vi "GetVarVal.vi"(8 "error in (no error)":errorcluster, 10 "varName":string, 11 "muExpr in":refnum<class "mupExpr.lvclass">) -> (0 "error out":errorcluster, 2 "varValue":dbl, 3 "muExpr out":refnum<class "mupExpr.lvclass">)   [LabVIEW 2018, in "mupExpr.lvclass"]
uses:
  mupExpr.lvclass
  mupExpr.lvclass/mupExpr.ctl
  <vilib>/Utility/error.llb/Error Cluster From Error Code.vi
  <vilib>/ErrorRing/Error Ring.xnode
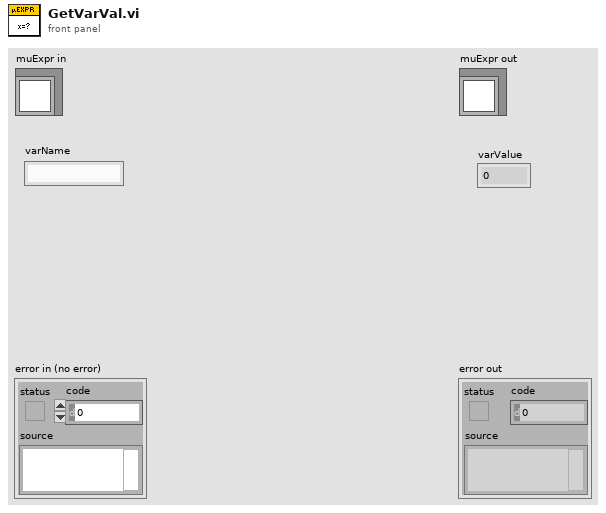
[diagram p1: front panel]
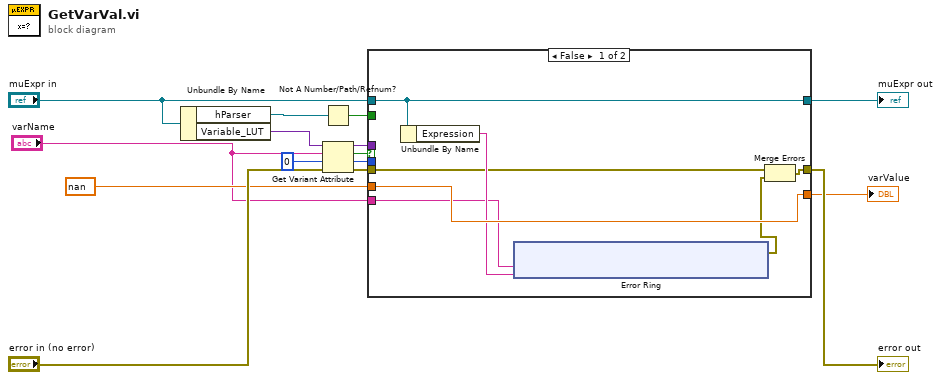
[diagram p0: block diagram]
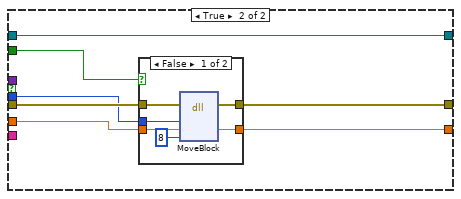
[diagram p2: hidden frame]
diagram:
  n1 = Unbundle By Name("muExpr in") -> ("hParser"=w2:refnum<data-value>, "Variable_LUT"=w8:variant)
  n2 = Not A Number/Path/Refnum?(number/path/refnum=w2) -> (NaN/Path/Refnum?=w1:bool)
  n3 = Get Variant Attribute(Variant=w8, name="varName", default value (empty Variant)=u64 0 ("pd"), error in="error in (no error)") -> (duplicate Variant=w3:variant, found=w4:bool, value=w5:u64, error out=w7:errorcluster)
  n4 = case shown="False" w4 {
    tunnel: w7 -> [w18 w36]
    tunnel: nan ("varValue") -> [w21 w34]
    tunnel: w5 -> [_ w33]
    tunnel: [w17 w35] -> w14
    tunnel: "varName" -> [w19 _]
    tunnel: "muExpr in" -> [w22 w37]
    tunnel: w3 -> [_ _]
    tunnel: [w22 w37] -> w12
    tunnel: [w21 w32] -> w9
    tunnel: w1 -> [_ w31]
    frame False {
      n5 = Unbundle By Name(w22) -> ("Expression"=w20:string)
      n6 = xnode "Error Ring"("parameter 0"=w19, "parameter 1"=w20) -> ("error out"=w16:errorcluster)
      n7 = Merge Errors(w18, w16) -> (w17:errorcluster)
    }
    frame True {
      n8 = case shown="False" w31 {
        tunnel: w36 -> [w42 w45]
        tunnel: [w41 w45] -> w35
        tunnel: w34 -> [w40 w44]
        tunnel: w33 -> [w39 _]
        tunnel: [w38 w44] -> w32
        frame False {
          n9 = dll-call lib="LabVIEW" fn="MoveBlock"(error in=w42, "ps"=w39, "pd"=w40, "size"=8) -> (error out=w41:errorcluster, "pd"=w38:dbl)  [unwired: 5 in, 1 out]
        }
        frame True {
        }
      }
    }
  }
  "error out" <- w14
  "muExpr out" <- w12
  "varValue" <- w9
